vi "GenOneOf_Get_Accessor.vi"(7 "application reference":refnum<vi>, 8 "error in (no error)":errorcluster, 10 "message element metadata":T1, 11 "path":path) -> (0 "error out":errorcluster)   [LabVIEW 2019, in "gRPC Template Creation Utility.lvlib"]
uses:
  gRPC Template Creation Utility.lvlib
  TypeDefs/Message Element Metadata (Scripting).ctl
  TypeDefs/Message Element Type.ctl
  <vilib>/Utility/traverseref.llb/TRef TravTarget.ctl
  <vilib>/Utility/traverseref.llb/VI Scripting - Traverse.lvlib
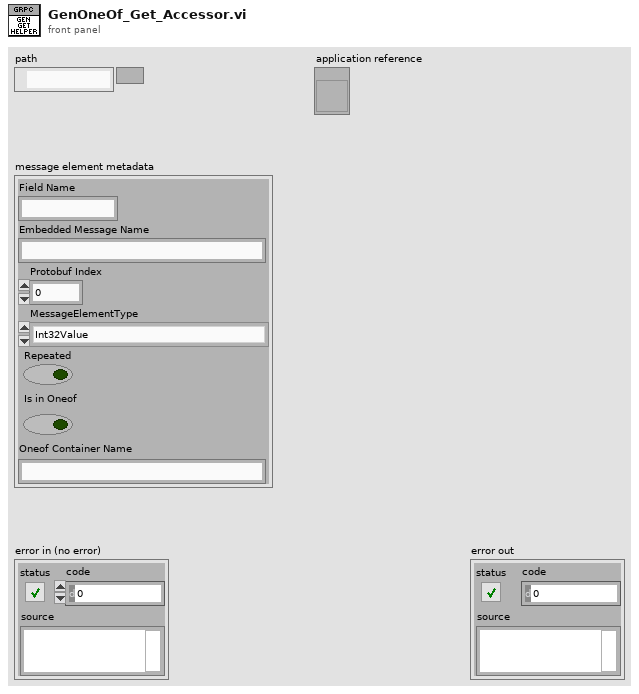
[diagram p1: front panel]
types:
  T1 = typedef "gRPC Template Creation Utility.lvlib/Message Element Metadata (Scripting).ctl" = cluster{"Field Name":string, "Embedded Message Name":string, "Protobuf Index":i32, "MessageElementType":T2, "Repeated":bool, "Is in Oneof":bool, "Oneof Container Name":string}
  T2 = typedef "gRPC Template Creation Utility.lvlib/Message Element Type.ctl" = enum32{"Int32Value", "FloatValue", "DoubleValue", "BoolValue", "StringValue", "MessageValue", "Int64Value", "UInt32Value", "UInt64Value", "EnumValue", "Bytes", "Fixed64", "Fixed32", "SFixed64", "SFixed32", "SInt64", "SInt32"}
  T3 = typedef "TRef TravTarget.ctl" = enum16{"FP", "BD", "Other"}
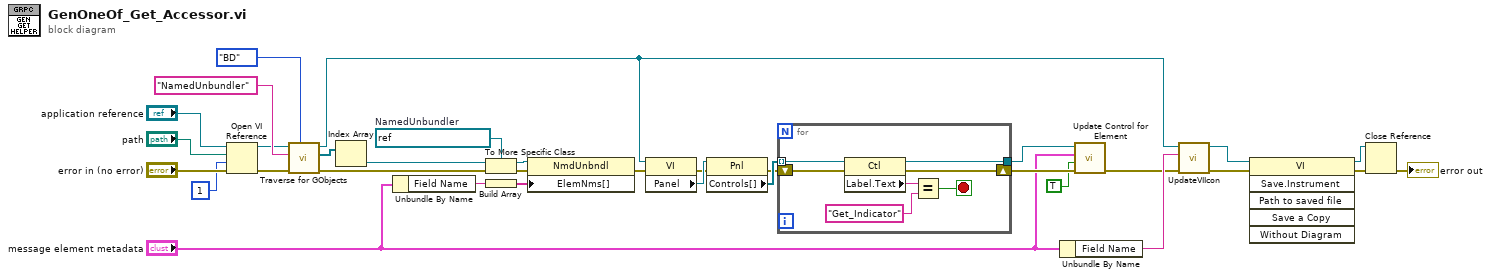
[diagram p0: block diagram]
diagram:
  w27 = refnum<vi> refnum  # NamedUnbundler
  n1 = Open VI Reference(application reference (local)="application reference", vi path="path", options=1, error in (no error)="error in (no error)") -> (vi reference=w22:refnum<vi>, error out=w13:errorcluster)  [unwired: 2 in]
  n2 = call <vilib>:"Traverse for GObjects.vi"("Traverse Target"=TRef_TravTarget."BD", "error in (no error)"=w13, "Class Name"="NamedUnbundler", "VI Refnum"=w22) -> ("error out"=w12:errorcluster, "References"=w28:refnum<vi>[], "dup VI Refnum"=w3:refnum<vi>)  [unwired: 4 in, 1 out]
  n3 = Index Array(array=w28) -> (element=w26:refnum<vi>)  [unwired: 1 in]
  n4 = Unbundle By Name("message element metadata") -> ("Field Name"=w7:string)
  n5 = To More Specific Class(target class=w27, reference=w26, error in=w12) -> (specific class reference=w23:refnum<vi>, error out=w19:errorcluster)
  n6 = Build Array(w7) -> (w25:string[])
  n7 = property class="NmdUnbndl"(reference=w23, error in=w19, "ElemNms[]"=w25) -> (error out=w18:errorcluster)  [unwired: 1 out]
  n8 = property class="VI"(reference=w3, error in=w18) -> (error out=w17:errorcluster, "Panel"=w21:refnum<vi>)  [unwired: 1 out]
  n9 = property class="Pnl"(reference=w21, error in=w17) -> (error out=w16:errorcluster, "Controls[]"=w20:refnum<vi>[])  [unwired: 1 out]
  n10 = for {
    tunnel: w20 -> [w40] mode=indexing
    tunnel: [w36] -> w10
    shift-right: [w34] -> w9
    shift-left: w16 -> [w35]
    stop <- w37 stop-if-true
    n11 = property class="Ctl"(reference=w40, error in=w35) -> (reference out=w36:refnum<vi>, error out=w34:errorcluster, "Label.Text"=w39:string)
    n12 = Equal?(x=w39, y="Get_Indicator") -> (x = y?=w37:bool)
  }
  n13 = Unbundle By Name("message element metadata") -> ("Field Name"=w6:string)
  n14 = call "Update Control for Element.vi"("error in (no error)"=w9, "indicator"=TRUE, "message element metadata"="message element metadata", "control to update"=w10) -> ("error out"=w5:errorcluster)  [unwired: 7 in]
  n15 = call "UpdateVIIcon.vi"("error in (no error)"=w5, "Method Name"=w6, "VI in"=w3) -> ("error out"=w4:errorcluster, "VI out"=w2:refnum<vi>)  [unwired: 7 in]
  n16 = invoke class="VI" method="Save.Instrument"(reference=w2, error in=w4) -> (reference out=w14:refnum<vi>, error out=w15:errorcluster)  [unwired: 4 in, 4 out]
  n17 = Close Reference(reference=w14, error in (no error)=w15) -> (error out=→"error out":errorcluster)
